vi "MDPtrMgr Sync.vi"(6 "timeout(10s)":u32=10, 8 "error in (no error)":errorcluster) -> (0 "error out":errorcluster, 1 "timeout?":bool, 4 "time esliped?":dbl)   [LabVIEW 2017, in "MDPtr.lvlib"]
uses:
  MDPtr.lvlib
  _MDPtrMgr/MDPtrMgr.lvclass
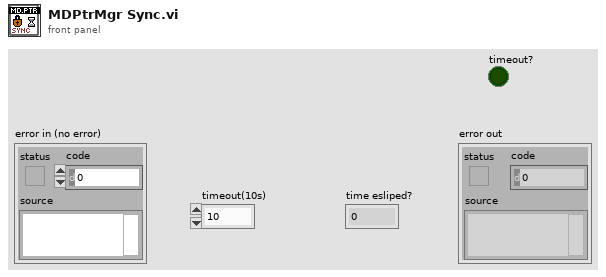
[diagram p1: front panel]
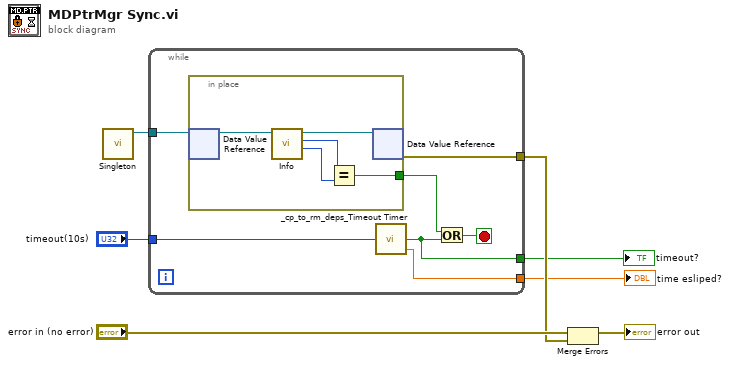
[diagram p0: block diagram]
diagram:
  n1 = call "Singleton.vi"() -> ("MDPtrMgrDVR"=w2:refnum<data-value>)  [unwired: 9 in, 2 out]
  n2 = while {
    tunnel: w2 -> [w14]
    tunnel: [w13] -> w5
    tunnel: "timeout(10s)" -> [w12]
    tunnel: [w9] -> w3
    tunnel: [w8] -> w1
    stop <- w10 stop-if-true
    n3 = in-place {
      in-place-border: [w15] -> w11
      n4 = in-place-dvr #1(w14) -> (w19:refnum<class "MDPtrMgr.lvclass">)  [unwired: 1 out]
      n5 = call "Info.vi"("MDPtrMgr in"=w19) -> ("# free MDPtrs in caches"=w16:i32, "# MDPtrs allocated"=w17:i32, "MDPtrMgr out"=w18:refnum<class "MDPtrMgr.lvclass">)  [unwired: 6 in, 2 out]
      n6 = Equal?(x=w17, y=w16) -> (x = y?=w15:bool)
      n7 = in-place-dvr #1(w18) -> (w13:errorcluster)  [unwired: 1 out]
    }
    n8 = call "_cp_to_rm_deps_Timeout Timer.vi"("timeout(s)"=w12) -> ("timeout?"=w9:bool, "time esliped?"=w8:dbl)  [unwired: 7 in]
    n9 = Or(x=w11, y=w9) -> (x .or. y?=w10:bool)
  }
  "timeout?" <- w3
  "time esliped?" <- w1
  n10 = Merge Errors("error in (no error)", w5) -> (→"error out":errorcluster)
